vi "Resource_Path.vi"(0 "File name":string, 5 "Subfolder":string="Levels", 11 "error in":errorcluster) -> (4 "Path":path, 15 "error out":errorcluster)   [LabVIEW 2020, in "GH_Level.lvlib"]
doc: "Absolute path of a file in the project: project folder\\Resources\\Subfolder\\File name. The project folder is derived from the path of this VI (Source\\Level)."
uses:
  GH_Level.lvlib
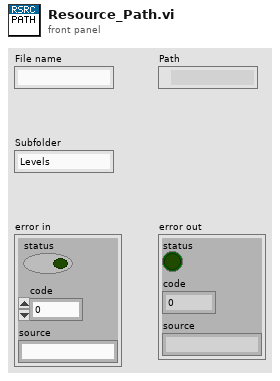
[diagram p1: front panel]
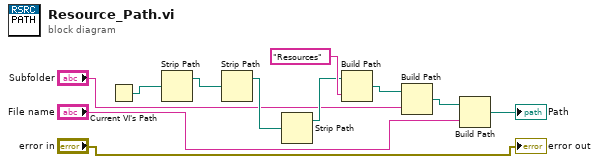
[diagram p0: block diagram]
diagram:
  n1 = Current VI's Path() -> (path=w4:path)
  n2 = Strip Path(path=w4) -> (stripped path=w5:path)  [unwired: 1 out]
  n3 = Strip Path(path=w5) -> (stripped path=w6:path)  [unwired: 1 out]
  n4 = Strip Path(path=w6) -> (stripped path=w7:path)  [unwired: 1 out]
  n5 = Build Path(base path=w7, name or relative path="Resources") -> (appended path=w9:path)
  n6 = Build Path(base path=w9, name or relative path="Subfolder") -> (appended path=w10:path)
  n7 = Build Path(base path=w10, name or relative path="File name") -> (appended path=→"Path":path)
  "error out" <- "error in"
